vi "protect ui.vi"() -> ()   [LabVIEW 2013, in "protection settings.lvclass"]
uses:
  protection settings.lvclass
  <vilib>/NI/Configuration Framework/Node/NodeRef.ctl
  <vilib>/NI/Configuration Framework/Node/NISE_CEF_Node.lvclass
  <vilib>/NI/AMC/Message Queue.ctl
  <vilib>/NI/AMC/Message.ctl
  <vilib>/NI/Tools/Keyed Array/KeyedArray.ctl
  <vilib>/NI/Configuration Framework/Node/UserEventRef.ctl
  <vilib>/NI/Configuration Framework/Controls/EventCluster.ctl
  protection settings.lvclass/protection settings.ctl
  Read Lock State.vi
  Read password.vi
  <vilib>/NI/Tools/Keyed Array/Tools_KeyedArray.lvlib
  <vilib>/NI/AMC/AMC.lvlib
  <vilib>/NI/Configuration Framework/NISE_CEF_TreeControl.lvlib
panel:
  in  "user event":T1
  in  "main queue":T2
  in  "node ref":T3
  in  "password (opt)":string
  in  "Lock State":T4(ring)=enum."Locked (No Password)"
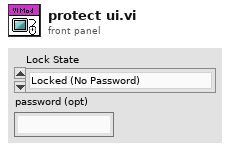
[diagram p1: front panel]
types:
  T1 = typedef "NISE_CEF_Node.lvclass/UserEventRef.ctl" = refnum<user-event>
  T2 = typedef "AMC.lvlib/Message Queue.ctl" = refnum<queue>
  T3 = typedef "NISE_CEF_Node.lvclass/NodeRef.ctl" = refnum<data-value>
  T4 = enum32{"invalid lock state", "Not Locked", "Locked (No Password)", "Password-protected"}
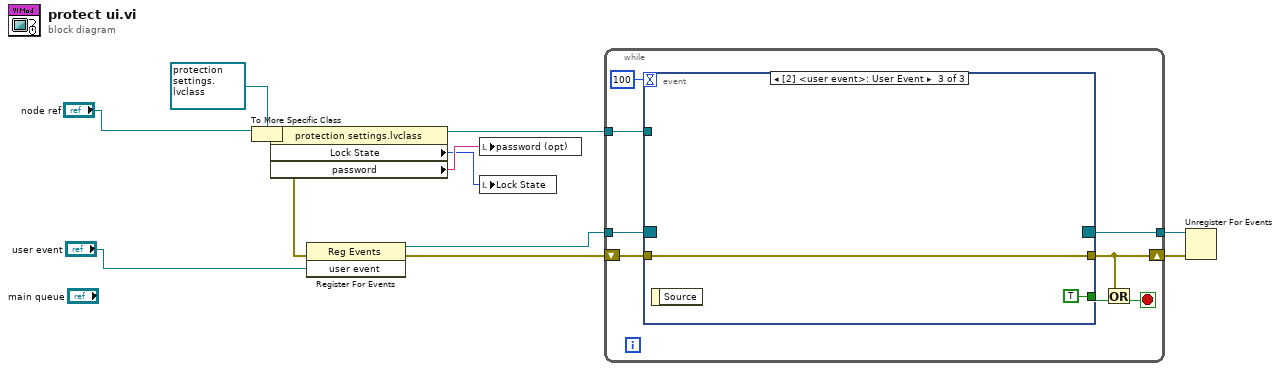
[diagram p0: block diagram]
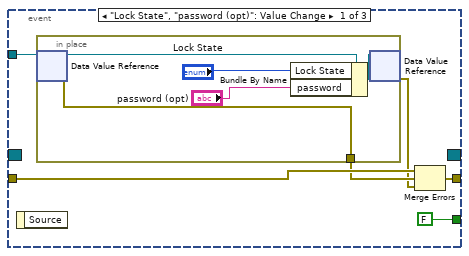
[diagram p2: hidden frame]
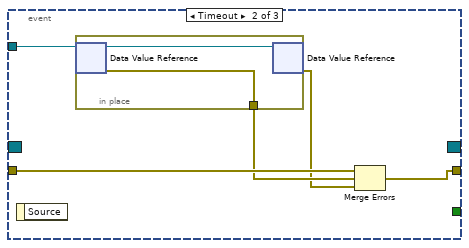
[diagram p3: hidden frame]
diagram:
  n1 = To More Specific Class(target class=refnum<data-value> refnum, reference="node ref") -> (specific class reference=w8:refnum<data-value>, error out=w6:errorcluster)  [unwired: 1 in]
  n2 = property class="protection settings.lvclass"(reference=w8) -> (reference out=w5:refnum<data-value>, "Lock State"=w3:T4, "password"=w4:string)  [unwired: 1 in, 1 out]
  n3 = register-events(error in=w6, "user event") -> (reference out=w11:refnum<event-registration>, error out=w12:errorcluster)  [unwired: 1 in]
  n4 = local write "password (opt)"(w4) -> ()
  n5 = local write "Lock State"(w3) -> ()
  n6 = while {
    shift-right: [w13] -> w10
    shift-left: w12 -> [w17]
    tunnel: w11 -> [w20]
    tunnel: [w19] -> w9
    tunnel: w5 -> [w16]
    stop <- w14 stop-if-true
    n7 = event shown="[2] <user event>: User Event" {
      selector: w20 -> [_ _ _]
      dyn-events: [_ _ _] -> w19
      timeout: 100 -> [_ _ _]
      tunnel: [FALSE _ TRUE] -> w18
      tunnel: [w24 w34 w40] -> w13
      tunnel: w17 -> [w26 w35 w40]
      tunnel: w16 -> [w25 w36 _]
      event "Lock State", "password (opt)": Value Change {
        n8 = event-data() -> ()  [unwired: 1 in, 1 out]
        n9 = in-place {
          in-place-border: [w29] -> w22
          n10 = in-place-dvr #1(w25) -> (w31:refnum<class "protection settings.lvclass">, w29:errorcluster)
          n11 = Bundle By Name(cluster=w31, "Lock State"="Lock State", "password"="password (opt)") -> (w30:refnum<class "protection settings.lvclass">)
          n12 = in-place-dvr #1(w30) -> (w21:errorcluster)  [unwired: 1 out]
        }
        n13 = Merge Errors(w26, w22, w21) -> (w24:errorcluster)
      }
      event Timeout {
        n14 = event-data() -> ()  [unwired: 1 in, 1 out]
        n15 = in-place {
          in-place-border: [w37] -> w33
          n16 = in-place-dvr #2(w36) -> (w38:refnum<class "protection settings.lvclass">, w37:errorcluster)
          n17 = in-place-dvr #2(w38) -> (w32:errorcluster)  [unwired: 1 out]
        }
        n18 = Merge Errors(w35, w33, w32) -> (w34:errorcluster)
      }
      event User Event {
        n19 = event-data() -> ()  [unwired: 1 in, 1 out]
      }
    }
    n20 = Or(x=w13, y=w18) -> (x .or. y?=w14:bool)
  }
  n21 = Unregister For Events(event registration refnum=w9, error in=w10) -> ()  [unwired: 1 out]
